vi "RT_Watchdog.vi"(8 "error in (no error)":errorcluster={"status"=FALSE, "code"=0, "source"="\"\""}, 10 "monotonic now":string, 11 "Heartbeat status":string) -> (0 "error out":errorcluster={"status"=FALSE, "code"=0, "source"="\"\""}, 2 "status ok":bool, 3 "Fault or controlled-shutdown request":string)   [LabVIEW 2026]
doc: "INTENT: Detect Host/executor heartbeat loss. LOGIC: Track sequence/elapsed deadlines and escalate loss to RT Fault Checker; keep local while Host fails."
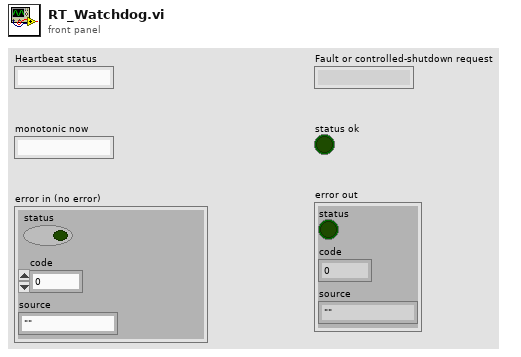
[diagram p1: front panel]
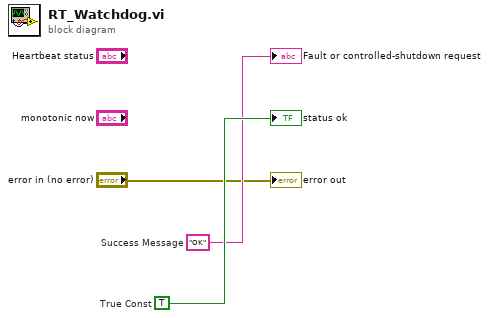
[diagram p0: block diagram]
diagram:
  w3 = TRUE  # True Const
  w2 = "OK"  # Success Message
  "Fault or controlled-shutdown request" <- w2
  "status ok" <- w3
  "error out" <- "error in (no error)"
